vi "N-664 Contol.vi"(0 "N-664 Notifier":refnum<notifier>, 5 "Stage Action":T1={"Action"=enum."Get Position", "Axis"=[], "Setpoint"=[], "Velocity"=0.5, "Cmd Recvd?"=FALSE, "Position"=[], "Status"=enum."Error", "Misc"=variant, "Servo On?"=FALSE} {"Velocity" min=0.0 max=1.0 step=0.01}, 11 "VISA In":refnum<visa-resource-name>) -> (4 "N-664 Notifier (Dup)":refnum<notifier>)   [LabVIEW 2016]
uses:
  Stages Controls/Stage Notifier Element.ctl
  Stages Controls/Stage Actions.ctl
  Stages Controls/Stage Status.ctl
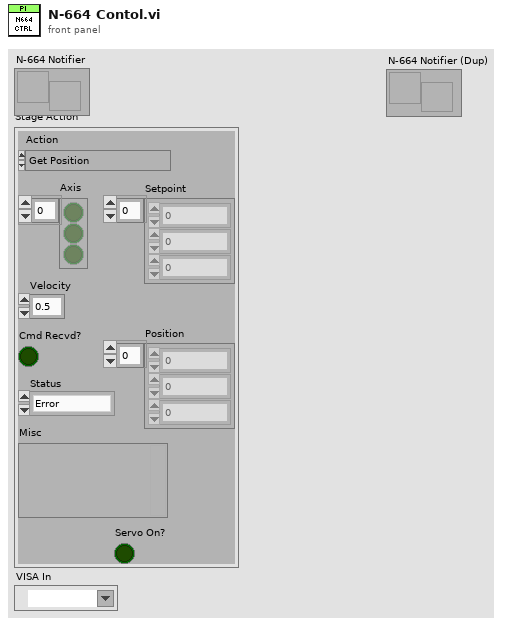
[diagram p1: front panel]
types:
  T1 = typedef "Stage Notifier Element.ctl" = cluster{"Action":T2, "Axis":bool[], "Setpoint":dbl[], "Velocity":dbl, "Cmd Recvd?":bool, "Position":dbl[], "Status":T3, "Misc":variant, "Servo On?":bool}
  T2 = typedef "Stage Actions.ctl" = enum16{"Get Position", "SERVO OFF", "SERVO ON", "SERVO ON/OFF", "MVR", "MOVE", "HALT", "ONTARGET", "ERROR", "REFERENCE", "INIT", "VELOCITY", "STATUS", "EXIT", "HOME", "ZEROPOS", "NANOPOS", "ANALOG", "QUIT"}
  T3 = typedef "Stage Status.ctl" = enum16{"Error", "Abort", "Busy", "On Target"}
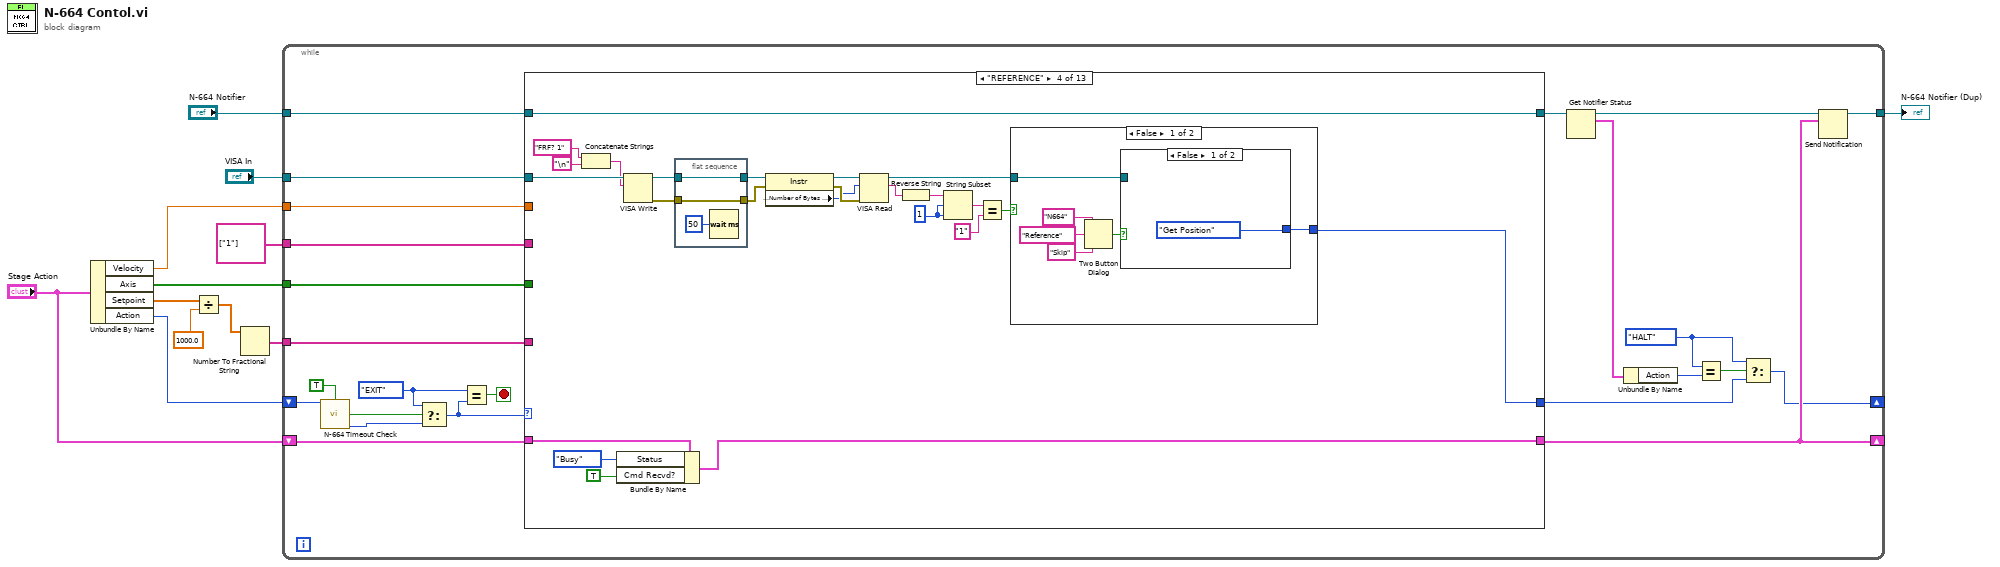
[diagram p0: block diagram]
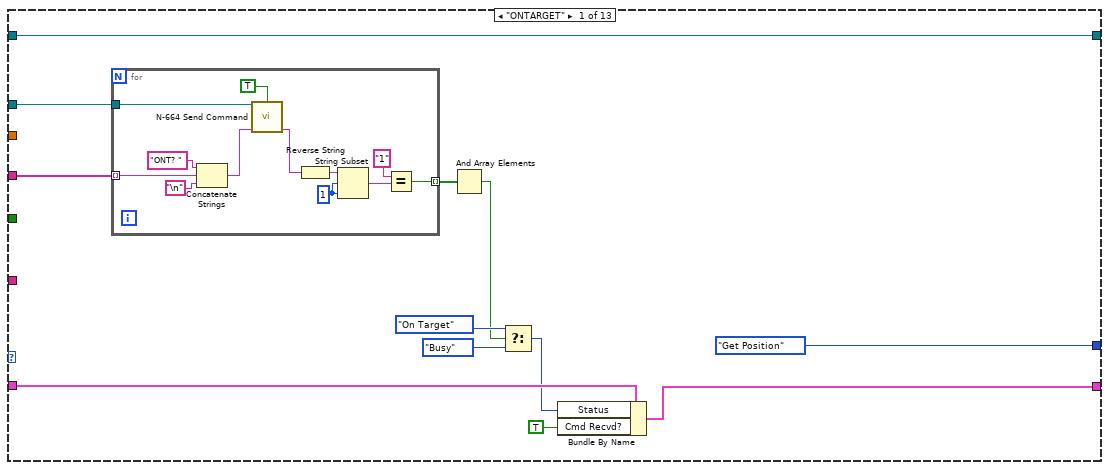
[diagram p2: hidden frame]
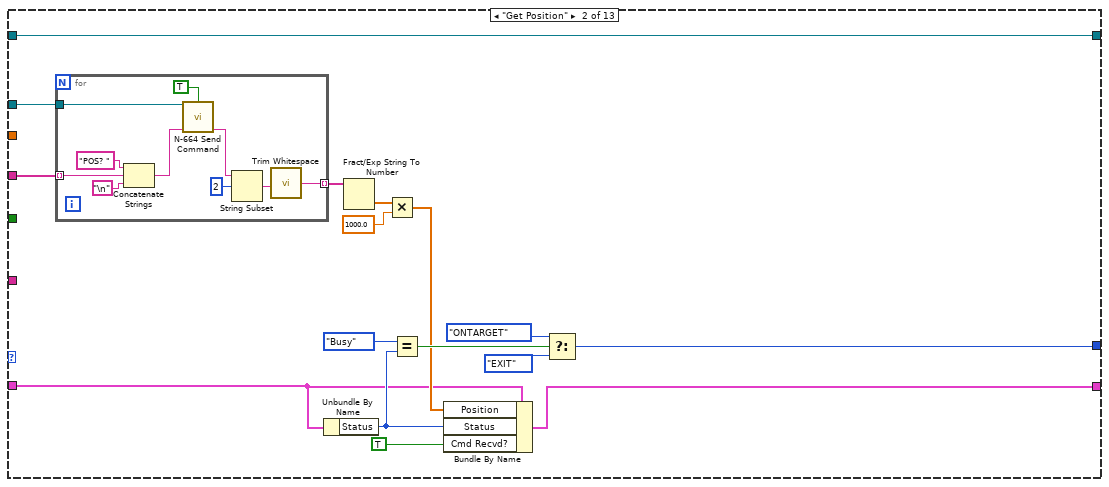
[diagram p3: hidden frame]
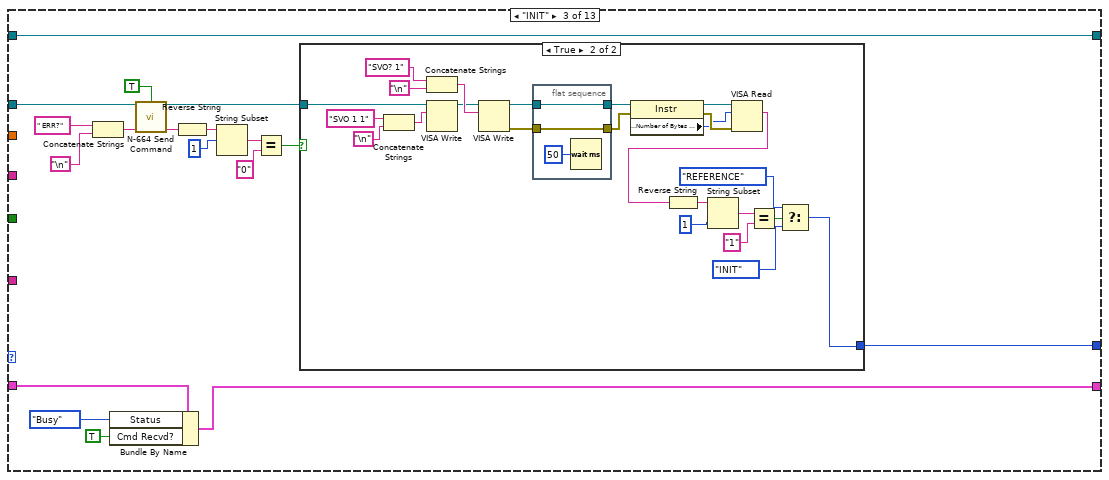
[diagram p4: hidden frame]
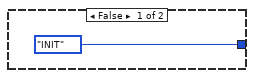
[diagram p5: hidden frame]
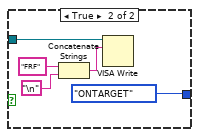
[diagram p6: hidden frame]
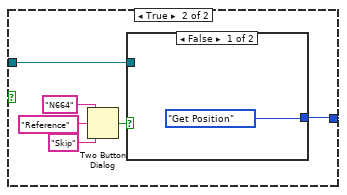
[diagram p7: hidden frame]
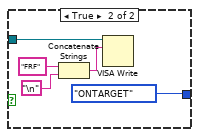
[diagram p8: hidden frame]
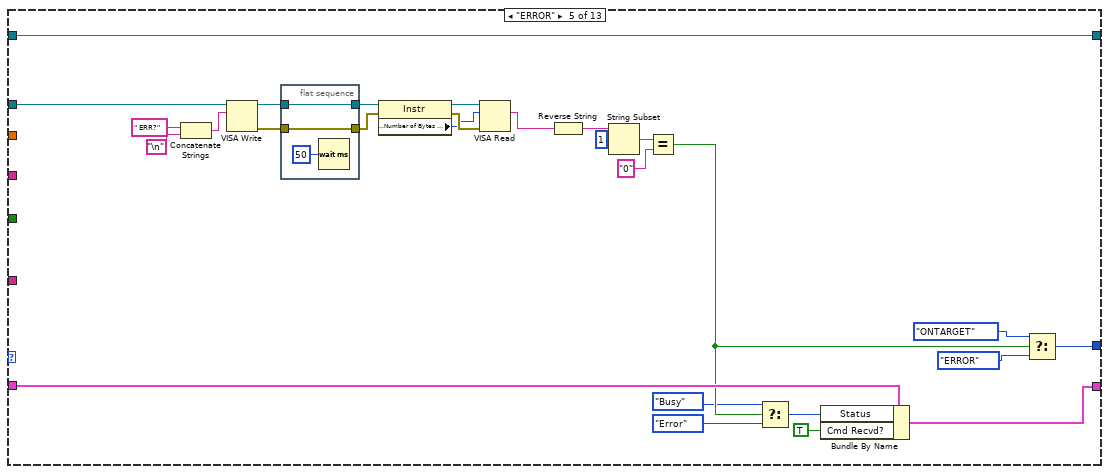
[diagram p9: hidden frame]
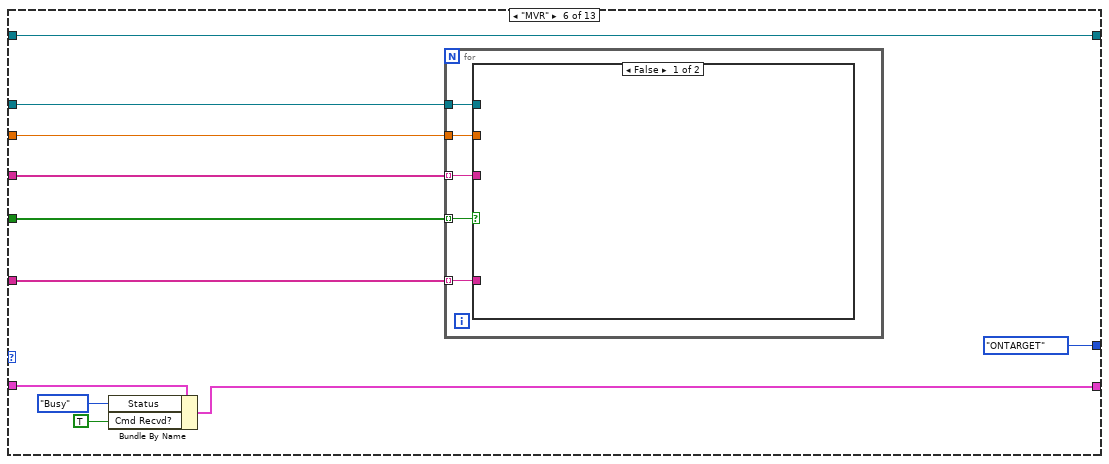
[diagram p10: hidden frame]
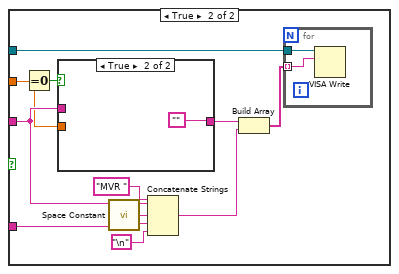
[diagram p11: hidden frame]
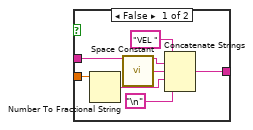
[diagram p12: hidden frame]
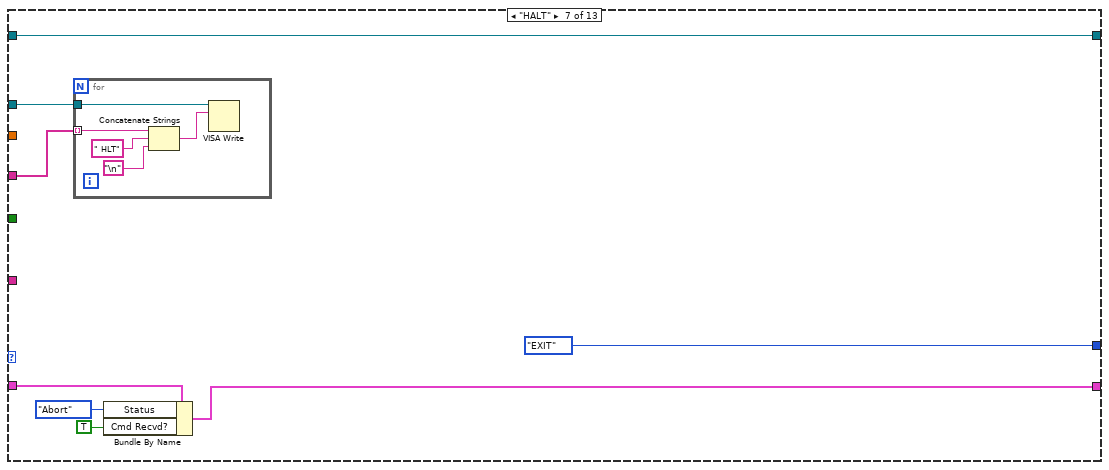
[diagram p13: hidden frame]
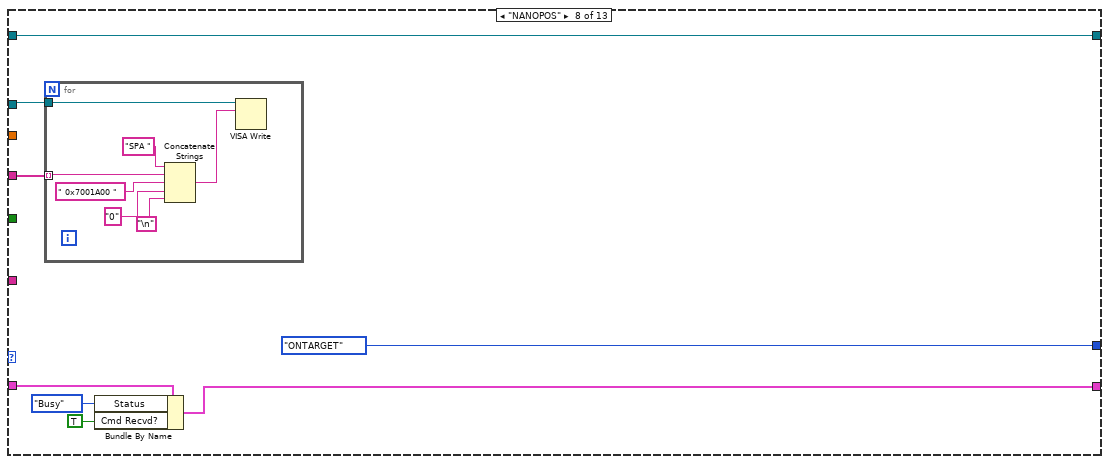
[diagram p14: hidden frame]
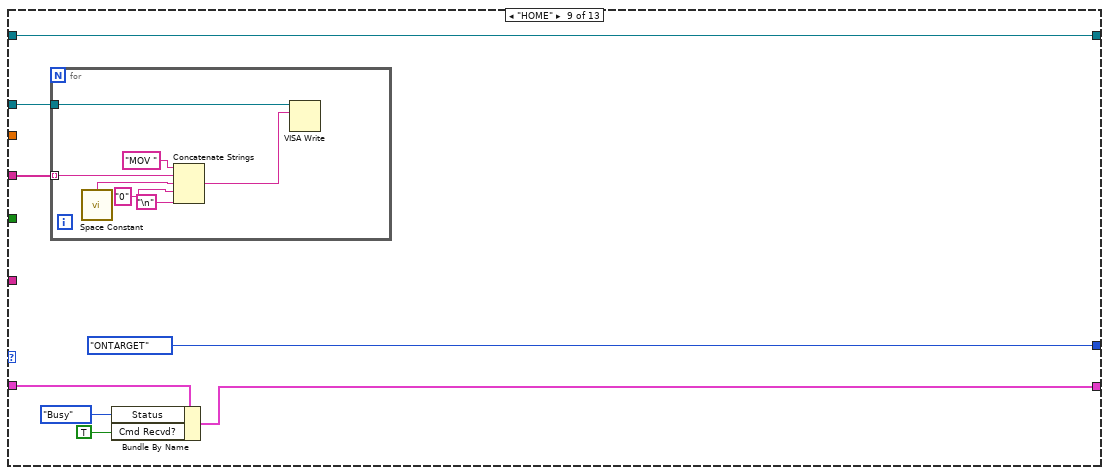
[diagram p15: hidden frame]
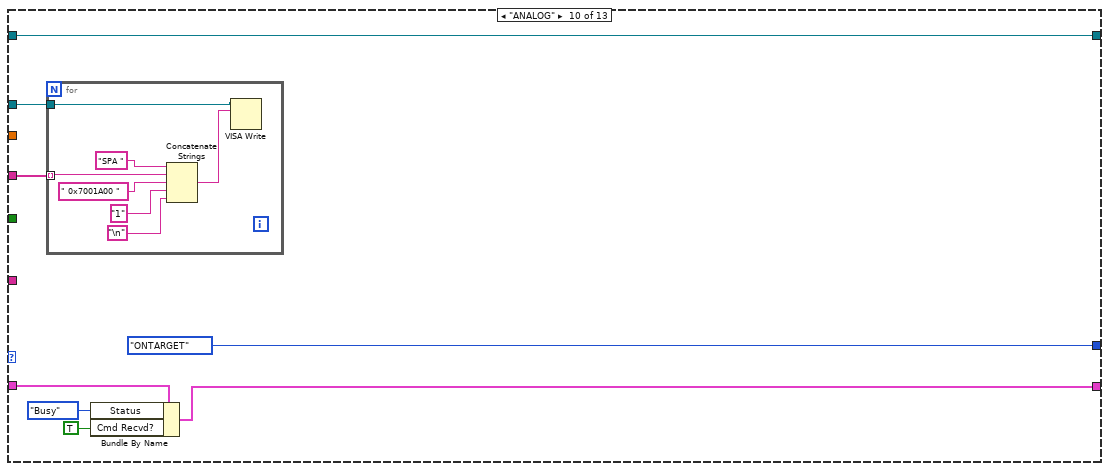
[diagram p16: hidden frame]
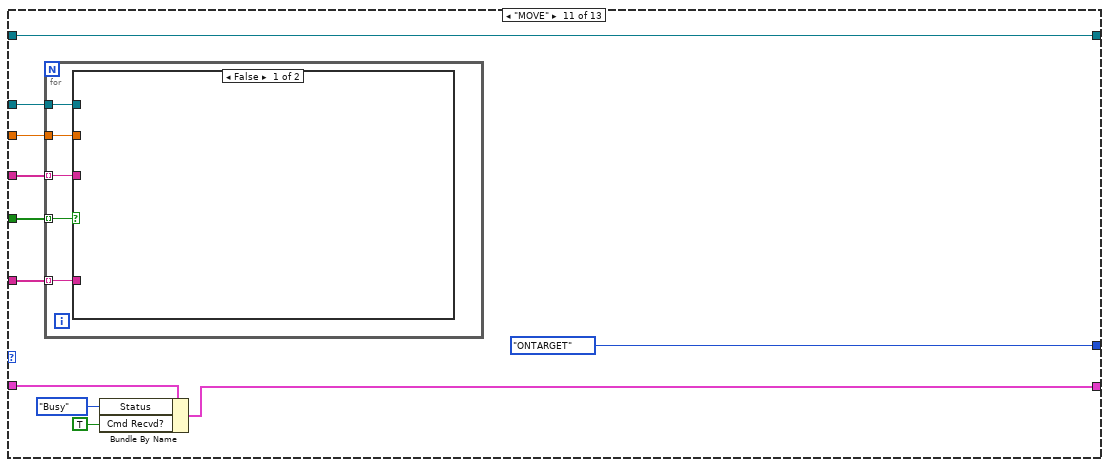
[diagram p17: hidden frame]
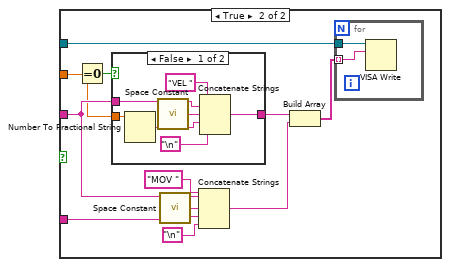
[diagram p18: hidden frame]
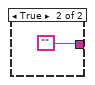
[diagram p19: hidden frame]
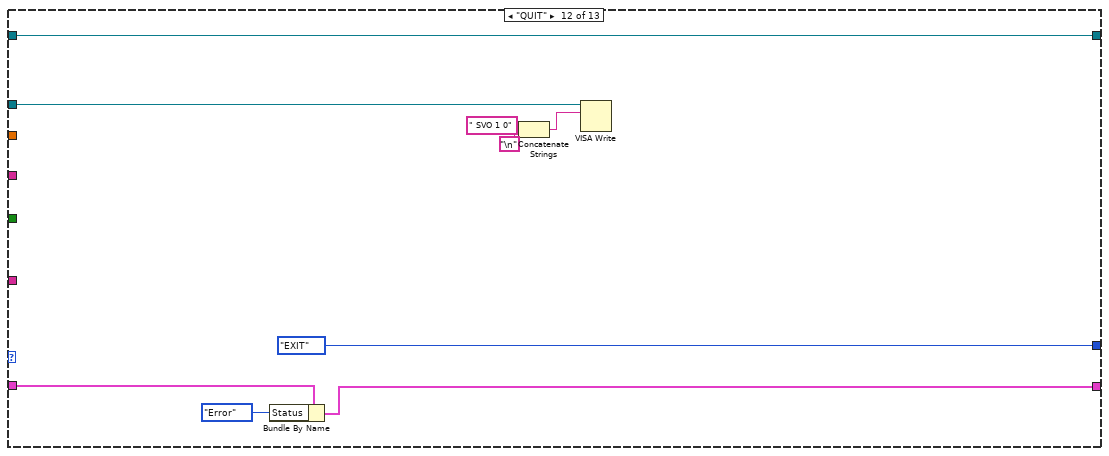
[diagram p20: hidden frame]
diagram:
  n1 = Unbundle By Name("Stage Action") -> ("Velocity"=w10:dbl, "Axis"=w9:bool[], "Setpoint"=w8:dbl[], "Action"=w7:T2)
  n2 = Divide(x=w8, y=1000.0) -> (x/y=w6:dbl[])
  n3 = Number To Fractional String(number=w6) -> (F-format string=w12:string[])  [unwired: 3 in]
  n4 = while {
    tunnel: string[] ["1"] -> [w36]
    shift-right: [w15] -> _
    shift-left: w7 -> [w28]
    tunnel: w9 -> [w34]
    tunnel: w10 -> [w33]
    tunnel: w12 -> [w35]
    shift-right: [w30] -> _
    shift-left: "Stage Action" -> [w32]
    tunnel: "N-664 Notifier" -> [w22]
    tunnel: "VISA In" -> [w14]
    tunnel: [w13] -> w1
    stop <- w23 stop-if-true
    w18 = Stage_Actions."HALT" ("Action")
    w27 = Stage_Actions."EXIT" ("t")
    n5 = call "N-664 Timeout Check.vi"("Action"=w28, "User Input?"=TRUE) -> ("Timeout?"=w26:bool, "Action (Dup)"=w25:T2)  [unwired: 12 in]
    n6 = Select(t=w27, s=w26, f=w25) -> (s? t:f=w24:T2)
    n7 = Equal?(x=w27, y=w24) -> (x = y?=w23:bool)
    n8 = case shown="\"REFERENCE\"" w24 {
      tunnel: w36 -> [w48 w76 _ _ _ w224 w258 w271 w286 w301 w319 _ _]
      tunnel: w14 -> [w37 w63 w92 w151 w188 w216 w252 w265 w280 w295 w309 w347 _]
      tunnel: w35 -> [_ _ _ _ _ w223 _ _ _ _ w318 _ _]
      tunnel: w34 -> [_ _ _ _ _ w222 _ _ _ _ w317 _ _]
      tunnel: w33 -> [_ _ _ _ _ w221 _ _ _ _ w316 _ _]
      tunnel: [Stage_Actions."Get Position" ("Action") w74 w104 w152 w204 Stage_Actions."ONTARGET" ("Action") Stage_Actions."EXIT" ("Action") Stage_Actions."ONTARGET" ("Action") Stage_Actions."ONTARGET" ("Action") Stage_Actions."ONTARGET" ("Action") Stage_Actions."ONTARGET" ("Action") Stage_Actions."EXIT" ("Action") Stage_Actions."EXIT" ("Action")] -> w31
      tunnel: w32 -> [w42 w61 w93 w154 w199 w218 w255 w268 w283 w298 w313 w353 w356]
      tunnel: [w38 w72 w101 w153 w201 w214 w254 w267 w282 w297 w312 w352 w356] -> w30
      tunnel: w22 -> [w39 w62 w87 w133 w184 w215 w251 w264 w279 w294 w310 w346 w355]
      tunnel: [w39 w62 w87 w133 w184 w215 w251 w264 w279 w294 w310 w346 w355] -> w17
      frame "ONTARGET" {
        n9 = for {
          tunnel: w48 -> [w60] mode=indexing
          tunnel: [w57] -> w47 mode=indexing
          tunnel: w37 -> [w52]
          w53 = 1 ("length (rest)")
          n10 = Concatenate Strings("ONT? " ("string"), w60, "\n") -> (w51:string)
          n11 = call "N-664 Send Command.vi"("VISA Ref"=w52, "Wait for Reply?"=TRUE, "Command"=w51) -> ("Response"=w50:string)  [unwired: 10 in, 2 out]
          n12 = Reverse String(1:w50) -> (0:w54:string)
          n13 = String Subset(string=w54, offset (0)=w53, length (rest)=w53) -> (substring=w59:string)
          n14 = Equal?(x="1", y=w59) -> (x = y?=w57:bool)
        }
        n15 = And Array Elements(Boolean array=w47) -> (logical AND=w43:bool)
        n16 = Select(t=Stage_Status."On Target" ("Status"), s=w43, f=Stage_Status."Busy" ("Status")) -> (s? t:f=w41:T3)
        n17 = Bundle By Name(cluster=w42, "Status"=w41, "Cmd Recvd?"=TRUE) -> (w38:T1)
      }
      frame "Get Position" {
        n18 = for {
          tunnel: w76 -> [w86] mode=indexing
          tunnel: [w85] -> w75 mode=indexing
          tunnel: w63 -> [w80]
          n19 = Concatenate Strings("POS? " ("string"), w86, "\n") -> (w78:string)
          n20 = call "N-664 Send Command.vi"("VISA Ref"=w80, "Wait for Reply?"=TRUE, "Command"=w78) -> ("Response"=w79:string)  [unwired: 10 in, 2 out]
          n21 = String Subset(string=w79, offset (0)=2) -> (substring=w81:string)  [unwired: 1 in]
          n22 = call <vilib>:"Trim Whitespace.vi"("string"=w81) -> ("trimmed string"=w85:string)  [unwired: 1 in]
        }
        n23 = Unbundle By Name(w61) -> ("Status"=w69:T3)
        n24 = Fract/Exp String To Number(string=w75) -> (number=w71:dbl[])  [unwired: 3 in, 1 out]
        n25 = Multiply(x=w71, y=1000.0) -> (x*y=w65:dbl[])
        n26 = Equal?(x=Stage_Status."Busy", y=w69) -> (x = y?=w68:bool)
        n27 = Bundle By Name(cluster=w61, "Position"=w65, "Status"=w69, "Cmd Recvd?"=TRUE) -> (w72:T1)
        n28 = Select(t=Stage_Actions."ONTARGET" ("Action"), s=w68, f=Stage_Actions."EXIT" ("Action")) -> (s? t:f=w74:T2)
      }
      frame "INIT" {
        n29 = Concatenate Strings(" ERR?" ("string"), "\n") -> (w89:string)
        n30 = Bundle By Name(cluster=w93, "Status"=Stage_Status."Busy", "Cmd Recvd?"=TRUE) -> (w101:T1)
        n31 = call "N-664 Send Command.vi"("VISA Ref"=w92, "Wait for Reply?"=TRUE, "Command"=w89) -> ("VISA Ref Out"=w91:refnum<visa-resource-name>, "Response"=w90:string)  [unwired: 10 in, 1 out]
        n32 = Reverse String(1:w90) -> (0:w97:string)
        n33 = String Subset(string=w97, offset (0)=1) -> (substring=w95:string)  [unwired: 1 in]
        n34 = Equal?(x=w95, y="0") -> (x = y?=w94:bool)
        n35 = case shown="True" w94 {
          tunnel: [Stage_Actions."INIT" ("Action") w106] -> w104
          tunnel: w91 -> [_ w121]
          frame False {
          }
          frame True {
            w126 = 1 ("length (rest)")
            n36 = Concatenate Strings("SVO 1 1" ("string"), "\n") -> (w128:string)
            n37 = Concatenate Strings("SVO? 1" ("string"), "\n") -> (w112:string)
            n38 = VISA Write(VISA resource name=w121, write buffer=w128) -> (VISA resource name out=w111:refnum<visa-resource-name>)  [unwired: 1 in, 2 out]
            n39 = VISA Write(VISA resource name=w111, write buffer=w112) -> (VISA resource name out=w119:refnum<visa-resource-name>, error out=w118:errorcluster)  [unwired: 1 in, 1 out]
            n40 = flat-sequence {
              tunnel: w119 -> [w131]
              tunnel: w118 -> [w130]
              tunnel: [w131] -> w117
              tunnel: [w130] -> w116
              frame #0 {
                n41 = Wait (ms)(milliseconds to wait=u32 50) -> ()  [unwired: 1 out]
              }
            }
            n42 = property class="Instr"(reference=w117, error in=w116) -> (reference out=w115:refnum<visa-resource-name>, error out=w114:errorcluster, "Serial Settings:Number of Bytes at Serial Port"=w113:u32)
            n43 = VISA Read(VISA resource name=w115, byte count=w113, error in (no error)=w114) -> (read buffer=w110:string)  [unwired: 3 out]
            n44 = Reverse String(1:w110) -> (0:w125:string)
            n45 = String Subset(string=w125, offset (0)=w126, length (rest)=w126) -> (substring=w123:string)
            n46 = Equal?(x=w123, y="1") -> (x = y?=w109:bool)
            n47 = Select(t=Stage_Actions."REFERENCE" ("Action"), s=w109, f=Stage_Actions."INIT" ("Action")) -> (s? t:f=w106:T2)
          }
        }
      }
      frame "REFERENCE" {
        w137 = 1 ("length (rest)")
        n48 = Concatenate Strings("FRF? 1" ("string"), "\n") -> (w141:string)
        n49 = Bundle By Name(cluster=w154, "Status"=Stage_Status."Busy", "Cmd Recvd?"=TRUE) -> (w153:T1)
        n50 = VISA Write(VISA resource name=w151, write buffer=w141) -> (VISA resource name out=w150:refnum<visa-resource-name>, error out=w149:errorcluster)  [unwired: 1 in, 1 out]
        n51 = flat-sequence {
          tunnel: w150 -> [w182]
          tunnel: w149 -> [w181]
          tunnel: [w182] -> w148
          tunnel: [w181] -> w147
          frame #0 {
            n52 = Wait (ms)(milliseconds to wait=u32 50) -> ()  [unwired: 1 out]
          }
        }
        n53 = property class="Instr"(reference=w148, error in=w147) -> (reference out=w146:refnum<visa-resource-name>, error out=w145:errorcluster, "Serial Settings:Number of Bytes at Serial Port"=w144:u32)
        n54 = VISA Read(VISA resource name=w146, byte count=w144, error in (no error)=w145) -> (VISA resource name out=w135:refnum<visa-resource-name>, read buffer=w136:string)  [unwired: 2 out]
        n55 = Reverse String(1:w136) -> (0:w138:string)
        n56 = String Subset(string=w138, offset (0)=w137, length (rest)=w137) -> (substring=w140:string)
        n57 = Equal?(x=w140, y="1") -> (x = y?=w134:bool)
        n58 = case shown="False" w134 {
          tunnel: [w158 w170] -> w152
          tunnel: w135 -> [w157 w169]
          frame False {
            n59 = Two Button Dialog(message="N664", 1:"Skip" ("F button name (\"Cancel\")"), 2:"Reference" ("T button name (\"OK\")")) -> (T button?=w159:bool)
            n60 = case shown="False" w159 {
              tunnel: [Stage_Actions."Get Position" ("Action") Stage_Actions."ONTARGET" ("Action")] -> w158
              tunnel: w157 -> [_ w164]
              frame False {
              }
              frame True {
                n61 = Concatenate Strings("FRF" ("string"), "\n") -> (w166:string)
                n62 = VISA Write(VISA resource name=w164, write buffer=w166) -> ()  [unwired: 1 in, 3 out]
              }
            }
          }
          frame True {
            n63 = Two Button Dialog(message="N664", 1:"Skip" ("F button name (\"Cancel\")"), 2:"Reference" ("T button name (\"OK\")")) -> (T button?=w171:bool)
            n64 = case shown="False" w171 {
              tunnel: [Stage_Actions."Get Position" ("Action") Stage_Actions."ONTARGET" ("Action")] -> w170
              tunnel: w169 -> [_ w176]
              frame False {
              }
              frame True {
                n65 = Concatenate Strings("FRF" ("string"), "\n") -> (w178:string)
                n66 = VISA Write(VISA resource name=w176, write buffer=w178) -> ()  [unwired: 1 in, 3 out]
              }
            }
          }
        }
      }
      frame "ERROR" {
        n67 = Concatenate Strings(" ERR?" ("string"), "\n") -> (w187:string)
        n68 = VISA Write(VISA resource name=w188, write buffer=w187) -> (VISA resource name out=w195:refnum<visa-resource-name>, error out=w194:errorcluster)  [unwired: 1 in, 1 out]
        n69 = flat-sequence {
          tunnel: w195 -> [w212]
          tunnel: w194 -> [w211]
          tunnel: [w212] -> w193
          tunnel: [w211] -> w192
          frame #0 {
            n70 = Wait (ms)(milliseconds to wait=u32 50) -> ()  [unwired: 1 out]
          }
        }
        n71 = property class="Instr"(reference=w193, error in=w192) -> (reference out=w191:refnum<visa-resource-name>, error out=w190:errorcluster, "Serial Settings:Number of Bytes at Serial Port"=w189:u32)
        n72 = VISA Read(VISA resource name=w191, byte count=w189, error in (no error)=w190) -> (read buffer=w186:string)  [unwired: 3 out]
        n73 = Reverse String(1:w186) -> (0:w207:string)
        n74 = String Subset(string=w207, offset (0)=1) -> (substring=w205:string)  [unwired: 1 in]
        n75 = Equal?(x=w205, y="0") -> (x = y?=w198:bool)
        n76 = Select(t=Stage_Status."Busy" ("Status"), s=w198, f=Stage_Status."Error" ("Status")) -> (s? t:f=w197:T3)
        n77 = Bundle By Name(cluster=w199, "Status"=w197, "Cmd Recvd?"=TRUE) -> (w201:T1)
        n78 = Select(t=Stage_Actions."ONTARGET" ("Action"), s=w198, f=Stage_Actions."ERROR") -> (s? t:f=w204:T2)
      }
      frame "MVR" {
        n79 = Bundle By Name(cluster=w218, "Status"=Stage_Status."Busy", "Cmd Recvd?"=TRUE) -> (w214:T1)
        n80 = for {
          tunnel: w224 -> [w229] mode=indexing
          tunnel: w223 -> [w228] mode=indexing
          tunnel: w222 -> [w227] mode=indexing
          tunnel: w221 -> [w226]
          tunnel: w216 -> [w225]
          n81 = case shown="False" w227 {
            tunnel: w229 -> [_ w236]
            tunnel: w228 -> [_ w237]
            tunnel: w225 -> [_ w230]
            tunnel: w226 -> [_ w235]
            frame False {
            }
            frame True {
              n82 = Equal To 0?(x=w235) -> (x = 0?=w234:bool)
              n83 = case shown="True" w234 {
                tunnel: w236 -> [w246 _]
                tunnel: w235 -> [w243 _]
                tunnel: [w245 ""] -> w233
                frame False {
                  n84 = Number To Fractional String(number=w243) -> (F-format string=w244:string)  [unwired: 3 in]
                  n85 = call <vilib>:"Space Constant.vi"() -> ("String"=w249:string)
                  n86 = Concatenate Strings("VEL ", w246, w249, w244, "\n") -> (w245:string)
                }
                frame True {
                }
              }
              n87 = call <vilib>:"Space Constant.vi"() -> ("String"=w238:string)
              n88 = Concatenate Strings("MVR ", w236, w238, w237, "\n") -> (w232:string)
              n89 = Build Array(w233, w232) -> (w231:string[])
              n90 = for {
                tunnel: w231 -> [w242] mode=indexing
                tunnel: w230 -> [w241]
                n91 = VISA Write(VISA resource name=w241, write buffer=w242) -> ()  [unwired: 1 in, 3 out]
              }
            }
          }
        }
      }
      frame "HALT" {
        n92 = for {
          tunnel: w258 -> [w260] mode=indexing
          tunnel: w252 -> [w259]
          n93 = Concatenate Strings(w260, " HLT" ("string"), "\n") -> (w261:string)
          n94 = VISA Write(VISA resource name=w259, write buffer=w261) -> ()  [unwired: 1 in, 3 out]
        }
        n95 = Bundle By Name(cluster=w255, "Status"=Stage_Status."Abort", "Cmd Recvd?"=TRUE) -> (w254:T1)
      }
      frame "NANOPOS" {
        n96 = for {
          tunnel: w271 -> [w275] mode=indexing
          tunnel: w265 -> [w272]
          n97 = Concatenate Strings("SPA " ("string"), w275, " 0x7001A00 " ("string"), "0", "\n") -> (w273:string)
          n98 = VISA Write(VISA resource name=w272, write buffer=w273) -> ()  [unwired: 1 in, 3 out]
        }
        n99 = Bundle By Name(cluster=w268, "Status"=Stage_Status."Busy", "Cmd Recvd?"=TRUE) -> (w267:T1)
      }
      frame "HOME" {
        n100 = for {
          tunnel: w286 -> [w289] mode=indexing
          tunnel: w280 -> [w287]
          n101 = call <vilib>:"Space Constant.vi"() -> ("String"=w290:string)
          n102 = Concatenate Strings("MOV " ("string"), w289, w290, "0" ("string"), "\n") -> (w288:string)
          n103 = VISA Write(VISA resource name=w287, write buffer=w288) -> ()  [unwired: 1 in, 3 out]
        }
        n104 = Bundle By Name(cluster=w283, "Status"=Stage_Status."Busy", "Cmd Recvd?"=TRUE) -> (w282:T1)
      }
      frame "ANALOG" {
        n105 = for {
          tunnel: w301 -> [w305] mode=indexing
          tunnel: w295 -> [w302]
          n106 = Concatenate Strings("SPA " ("string"), w305, " 0x7001A00 " ("string"), "1", "\n") -> (w304:string)
          n107 = VISA Write(VISA resource name=w302, write buffer=w304) -> ()  [unwired: 1 in, 3 out]
        }
        n108 = Bundle By Name(cluster=w298, "Status"=Stage_Status."Busy", "Cmd Recvd?"=TRUE) -> (w297:T1)
      }
      frame "MOVE" {
        n109 = for {
          tunnel: w319 -> [w324] mode=indexing
          tunnel: w318 -> [w323] mode=indexing
          tunnel: w317 -> [w322] mode=indexing
          tunnel: w316 -> [w321]
          tunnel: w309 -> [w320]
          n110 = case shown="False" w322 {
            tunnel: w324 -> [_ w331]
            tunnel: w323 -> [_ w332]
            tunnel: w320 -> [_ w325]
            tunnel: w321 -> [_ w330]
            frame False {
            }
            frame True {
              n111 = Equal To 0?(x=w330) -> (x = 0?=w329:bool)
              n112 = case shown="False" w329 {
                tunnel: w331 -> [w341 _]
                tunnel: w330 -> [w338 _]
                tunnel: [w340 ""] -> w328
                frame False {
                  n113 = Number To Fractional String(number=w338) -> (F-format string=w339:string)  [unwired: 3 in]
                  n114 = call <vilib>:"Space Constant.vi"() -> ("String"=w344:string)
                  n115 = Concatenate Strings("VEL ", w341, w344, w339, "\n") -> (w340:string)
                }
                frame True {
                }
              }
              n116 = call <vilib>:"Space Constant.vi"() -> ("String"=w333:string)
              n117 = Concatenate Strings("MOV ", w331, w333, w332, "\n") -> (w327:string)
              n118 = Build Array(w328, w327) -> (w326:string[])
              n119 = for {
                tunnel: w326 -> [w337] mode=indexing
                tunnel: w325 -> [w336]
                n120 = VISA Write(VISA resource name=w336, write buffer=w337) -> ()  [unwired: 1 in, 3 out]
              }
            }
          }
        }
        n121 = Bundle By Name(cluster=w313, "Status"=Stage_Status."Busy", "Cmd Recvd?"=TRUE) -> (w312:T1)
      }
      frame "QUIT" {
        n122 = Bundle By Name(cluster=w353, "Status"=Stage_Status."Error") -> (w352:T1)
        n123 = Concatenate Strings(" SVO 1 0" ("string"), "\n") -> (w350:string)
        n124 = VISA Write(VISA resource name=w347, write buffer=w350) -> ()  [unwired: 1 in, 3 out]
      }
      frame "EXIT", Default {
      }
    }
    n125 = Get Notifier Status(notifier=w17) -> (notifier out=w21:refnum<notifier>, current notification=w16:T1)  [unwired: 1 in, 3 out]
    n126 = Unbundle By Name(w16) -> ("Action"=w19:T2)
    n127 = Equal?(x=w18, y=w19) -> (x = y?=w20:bool)
    n128 = Select(t=w18, s=w20, f=w31) -> (s? t:f=w15:T2)
    n129 = Send Notification(notification=w30, notifier=w21) -> (notifier out=w13:refnum<notifier>)  [unwired: 1 in, 1 out]
  }
  "N-664 Notifier (Dup)" <- w1
